vi "C_RX_Buffers_Init.vi"(8 "error in (no error)":errorcluster) -> (0 "error out":errorcluster, 1 "pcap":u8[](array[numeric]), 2 "tx":u8[](array[numeric]), 3 "buffers":T1)   [LabVIEW 2021, in "CANsub_C.lvlib"]
doc: "Allocates every receive buffer once (frame arrays for 1756 frames, both decoder states, ping), the 174-byte tx buffer and the pcap buffer, and runs the library warm-up, so the real-time loop has no allocation and no page faults. Call once before the loop; keep buffers, tx and pcap in shift registers."
uses:
  CANsub_C.lvlib
  C_RX_Buffers.ctl
  codec_vis/CANsub_Codec.lvlib
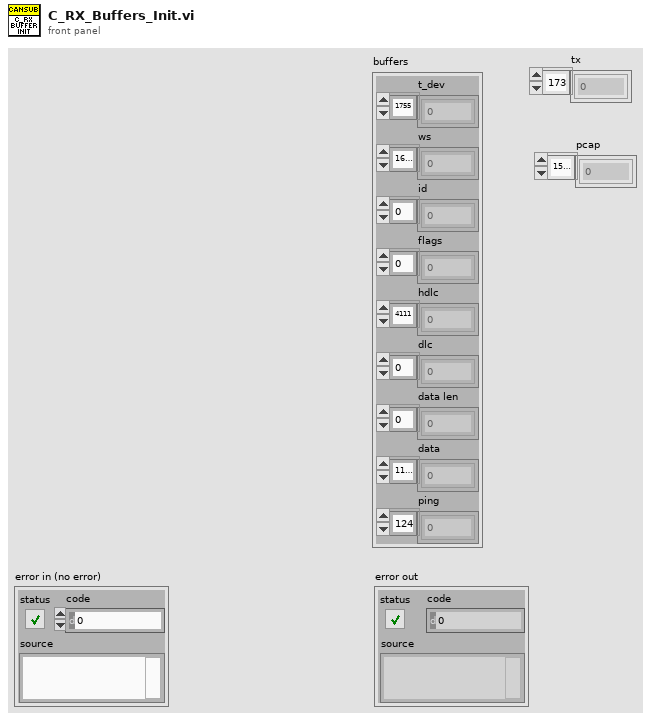
[diagram p1: front panel]
types:
  T1 = typedef "CANsub_C.lvlib/C_RX_Buffers.ctl" = cluster{"t_dev":dbl[], "ws":u8[], "id":u32[], "flags":u16[], "hdlc":u8[], "dlc":u8[], "data len":u8[], "data":u8[], "ping":u8[]}
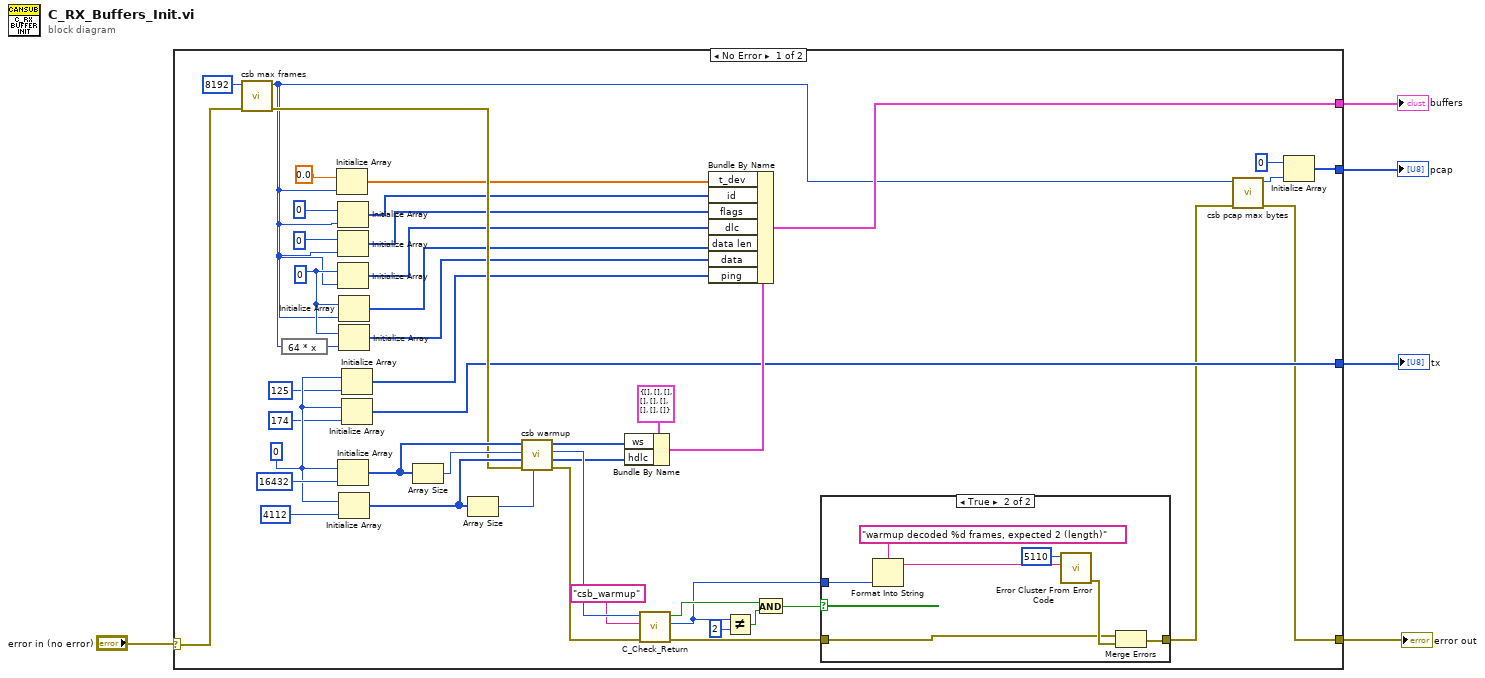
[diagram p0: block diagram]
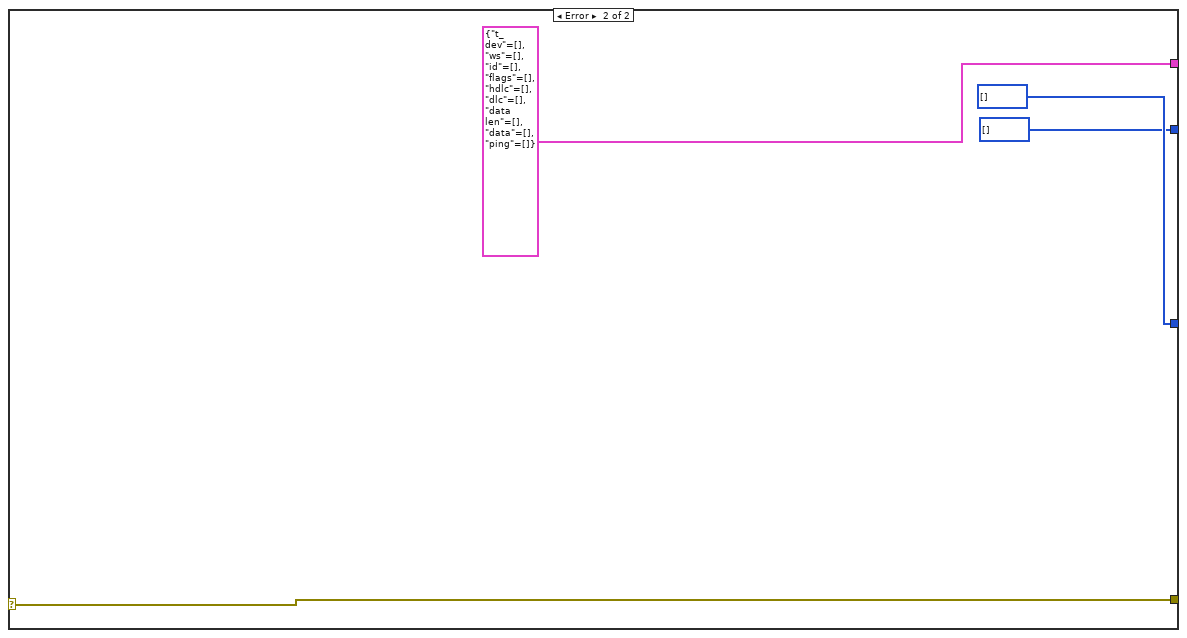
[diagram p3: hidden frame]
diagram:
  n1 = case shown="No Error" "error in (no error)" {
    selector: "error in (no error)" -> [w32 w62]
    tunnel: [w6 w62] -> w4
    tunnel: [w12 T1 {"t_dev"=[], "ws"=[], "id"=[], "flags"=[], "hdlc"=[], "dlc"=[], "data len"=[], "data"=[], "ping"=[]} ("buffers")] -> w3
    tunnel: [w20 u8[] [] ("tx")] -> w2
    tunnel: [w8 u8[] [] ("pcap")] -> w1
    frame No Error {
      w44 = u8 0
      w47 = u8 0
      n2 = call "csb max frames.vi"("error in (no error)"=w32, "in_len"=8192) -> ("error out"=w31:errorcluster, "function return"=w11:i32)  [unwired: 8 in]
      n3 = expression code="64 * x"(w11) -> (w40:i32)
      n4 = Initialize Array(0.0, w11) -> (w13:dbl[])
      n5 = Initialize Array(u32 0, w11) -> (w14:u32[])
      n6 = Initialize Array(u16 0, w11) -> (w15:u16[])
      n7 = Initialize Array(w44, w11) -> (w16:u8[])
      n8 = Initialize Array(w47, 16432 ("dimension size")) -> (w37:u8[])
      n9 = Initialize Array(w44, w11) -> (w17:u8[])
      n10 = Initialize Array(w44, w40) -> (w18:u8[])
      n11 = Initialize Array(w47, 4112 ("dimension size")) -> (w35:u8[])
      n12 = Initialize Array(w47, 125 ("dimension size")) -> (w19:u8[])
      n13 = Initialize Array(w47, 174 ("dimension size")) -> (w20:u8[])
      n14 = Array Size(array=w37) -> (size(s)=w36:i32)
      n15 = Array Size(array=w35) -> (size(s)=w34:i32)
      n16 = call "csb warmup.vi"("hdlc_state_size"=w34, "error in (no error)"=w31, "hdlc_state"=w35, "ws_state_size"=w36, "ws_state"=w37) -> ("error out"=w33:errorcluster, "hdlc_state out"=w28:u8[], "function return"=w39:i32, "ws_state out"=w29:u8[])  [unwired: 3 in]
      n17 = Bundle By Name(cluster=T1 {"t_dev"=[], "ws"=[], "id"=[], "flags"=[], "hdlc"=[], "dlc"=[], "data len"=[], "data"=[], "ping"=[]} ("C_RX_Buffers"), "ws"=w29, "hdlc"=w28) -> (w21:T1)
      n18 = call "C_Check_Return.vi"("error in (no error)"=w33, "function name"="csb_warmup", "function return"=w39) -> ("error out"=w23:errorcluster, "length"=w22:i32, "ok"=w25:bool)  [unwired: 6 in]
      n19 = Bundle By Name(cluster=w21, "t_dev"=w13, "id"=w14, "flags"=w15, "dlc"=w16, "data len"=w17, "data"=w18, "ping"=w19) -> (w12:T1)
      n20 = Not Equal?(x=w22, y=2) -> (x != y?=w24:bool)
      n21 = And(x=w25, y=w24) -> (x .and. y?=w27:bool)
      n22 = case shown="True" w27 {
        tunnel: [w51 w52] -> w7
        tunnel: w23 -> [w51 w53]
        tunnel: w22 -> [_ w56]
        frame False {
        }
        frame True {
          n23 = Format Into String(format string="warmup decoded %d frames, expected 2 (length)", w56) -> (resulting string=w55:string)  [unwired: 2 in, 1 out]
          n24 = call <vilib>:"Error Cluster From Error Code.vi"("error message (\"\")"=w55, "error code (0)"=5110) -> ("error out"=w54:errorcluster)  [unwired: 7 in]
          n25 = Merge Errors(w53, w54) -> (w52:errorcluster)
        }
      }
      n26 = call "csb pcap max bytes.vi"("error in (no error)"=w7, "n_frames"=w11) -> ("error out"=w6:errorcluster, "function return"=w10:i32)  [unwired: 8 in]
      n27 = Initialize Array(u8 0, w10) -> (w8:u8[])
    }
    frame Error {
    }
  }
  "error out" <- w4
  "buffers" <- w3
  "tx" <- w2
  "pcap" <- w1
